vi "ProgressWindow.vi"(0 "ClassWriter in":refnum<class "ClassWriter.lvclass">, 1 "Message(Exit)":string="Exit", 5 "error in (no error)":errorcluster) -> (14 "ClassWriter out":refnum<class "ClassWriter.lvclass">, 19 "error out":errorcluster)   [LabVIEW 2020, in "ClassWriter.lvclass"]
uses:
  ClassWriter.lvclass
  ClassWriter.lvclass/ClassWriter.ctl
  ProgressWindowDialog.vi
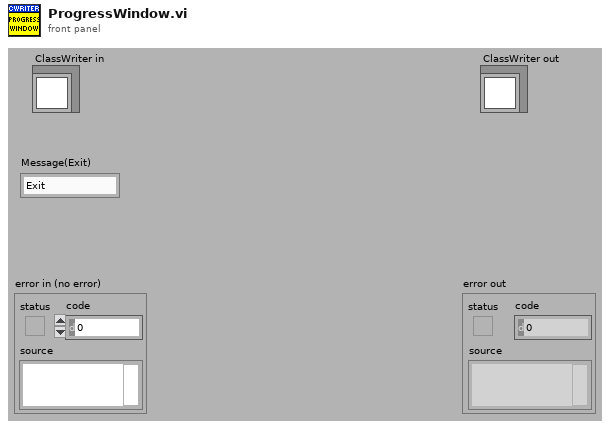
[diagram p1: front panel]
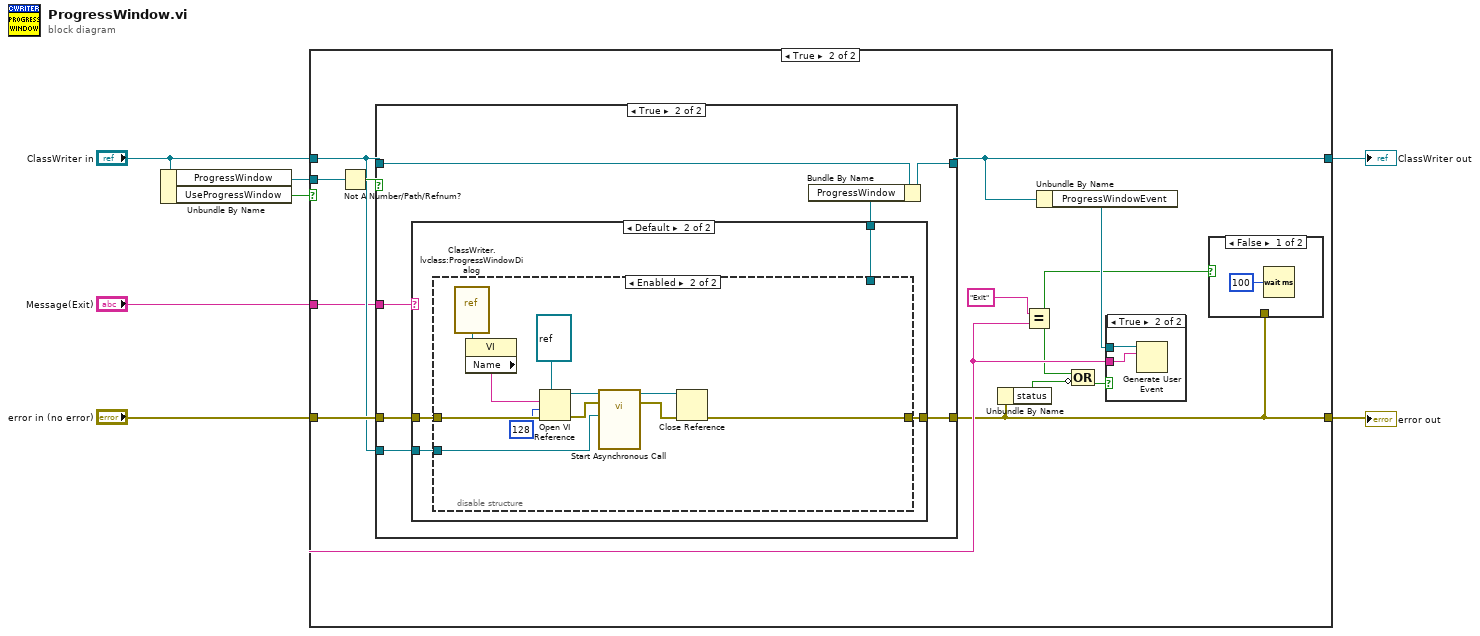
[diagram p0: block diagram]
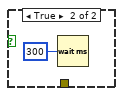
[diagram p4: hidden frame]
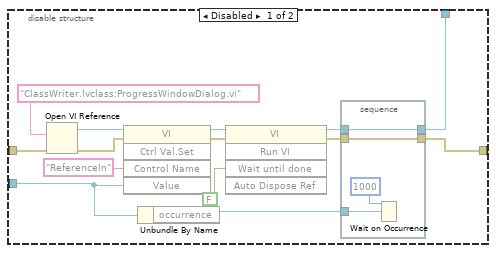
[diagram p7: hidden frame]
diagram:
  n1 = Unbundle By Name("ClassWriter in") -> ("ProgressWindow"=w7:refnum<vi>, "UseProgressWindow"=w1:bool)
  n2 = case shown="True" w1 {
    tunnel: w7 -> [_ w21]
    tunnel: "error in (no error)" -> [w9 w19]
    tunnel: [w8 w18] -> w5
    tunnel: "ClassWriter in" -> [w8 w16]
    tunnel: "Message(Exit)" -> [_ w15]
    tunnel: [w9 w13] -> w2
    frame False {
    }
    frame True {
      n3 = Not A Number/Path/Refnum?(number/path/refnum=w21) -> (NaN/Path/Refnum?=w20:bool)
      n4 = case shown="True" w20 {
        tunnel: w19 -> [w26 w34]
        tunnel: w16 -> [_ w33]
        tunnel: w16 -> [w27 w32]
        tunnel: [w27 w31] -> w18
        tunnel: [w26 w29] -> w13
        tunnel: w15 -> [_ w28]
        frame False {
        }
        frame True {
          n5 = case shown="Default" w28 {
            tunnel: w34 -> [w35 w39]
            tunnel: w33 -> [_ w36]
            tunnel: [_ w38] -> w30
            tunnel: [w35 w37] -> w29
            frame "Exit", "Hide", "UnHide" {
            }
            frame Default {
              n6 = disable-structure shown="Enabled" {
                disable-tunnel: w39 -> [w53 w67]
                disable-tunnel: [w44 _] -> w38
                disable-tunnel: [w43 w60] -> w37
                disable-tunnel: w36 -> [w40 w62]
                frame Disabled {
                  n7 = Open VI Reference(vi path="ClassWriter.lvclass:ProgressWindowDialog.vi", error in (no error)=w53) -> (vi reference=w41:refnum<vi>, error out=w51:errorcluster)  [unwired: 4 in]
                  n8 = invoke class="VI" method="Ctrl Val.Set"(reference=w41, error in=w51, "Control Name"="ReferenceIn", "Value"=w40) -> (reference out=w49:refnum<vi>, error out=w48:errorcluster)  [unwired: 1 in, 3 out]
                  n9 = Unbundle By Name(w40) -> ("occurrence"=w47:refnum<k4>)
                  n10 = invoke class="VI" method="Run VI"(reference=w49, error in=w48, "Wait until done"=FALSE ("Wait Until Done")) -> (reference out=w46:refnum<vi>, error out=w45:errorcluster)  [unwired: 2 in, 3 out]
                  n11 = stacked-sequence {
                    tunnel: w47 -> [w55]
                    tunnel: w46 -> [w57]
                    tunnel: w45 -> [w56]
                    tunnel: [w57] -> w44
                    tunnel: [w56] -> w43
                    frame #0 {
                      n12 = Wait on Occurrence(2:w55, 3:1000 ("ms timeout (-1)")) -> ()  [unwired: 1 in, 1 out]
                    }
                  }
                }
                frame Enabled {
                  n13 = vi-ref "ClassWriter.lvclass:ProgressWindowDialog.vi"() -> (w68:refnum<vi>)
                  n14 = property class="VI"(reference=w68) -> ("Name"=w65:string)  [unwired: 1 in, 2 out]
                  n15 = Open VI Reference(type specifier VI Refnum (for type only)=refnum<vi> refnum, vi path=w65, options=128, error in (no error)=w67) -> (vi reference=w64:refnum<vi>, error out=w63:errorcluster)  [unwired: 2 in]
                  n16 = call-by-ref "Start Asynchronous Call"(reference=w64, error in=w63, "ReferenceIn"=w62) -> (reference out=w61:refnum<vi>, error out=w59:errorcluster)  [unwired: 18 in, 1 out]
                  n17 = Close Reference(reference=w61, error in (no error)=w59) -> (error out=w60:errorcluster)
                }
              }
            }
          }
          n18 = Bundle By Name(cluster=w32, "ProgressWindow"=w30) -> (w31:refnum<class "ClassWriter.lvclass">)
        }
      }
      n19 = Unbundle By Name(w13) -> ("status"=w12:bool)
      n20 = Equal?(x="Exit", y=w15) -> (x = y?=w10:bool)
      n21 = Unbundle By Name(w18) -> ("ProgressWindowEvent"=w17:refnum<user-event>)
      n22 = Compound Arithmetic op=OR(w10, invert w12) -> (w11:bool)
      n23 = case shown="True" w11 {
        tunnel: w17 -> [_ w23]
        tunnel: w15 -> [_ w22]
        frame False {
        }
        frame True {
          n24 = Generate User Event(user event=w23, event data cluster=w22) -> ()  [unwired: 2 in, 2 out]
        }
      }
      n25 = case shown="False" w10 {
        tunnel: w13 -> [_ _]
        frame False {
          n26 = Wait (ms)(milliseconds to wait=u32 100) -> ()  [unwired: 1 out]
        }
        frame True {
          n27 = Wait (ms)(milliseconds to wait=u32 300) -> ()  [unwired: 1 out]
        }
      }
    }
  }
  "error out" <- w2
  "ClassWriter out" <- w5
